vi "Unload.vi"(8 "error in (no error)":errorcluster, 10 "Unload":string, 11 "Sequencing in":refnum<class "Sequencing.lvclass">) -> (0 "error out":errorcluster, 3 "Sequencing out":refnum<class "Sequencing.lvclass">)   [LabVIEW 2020, in "VolatusSeq.lvlib" / "Sequencing.lvclass"]
uses:
  Sequencing.lvclass
  Sequencing.lvclass/Sequencing.ctl
  Sequence/Sequence.lvclass
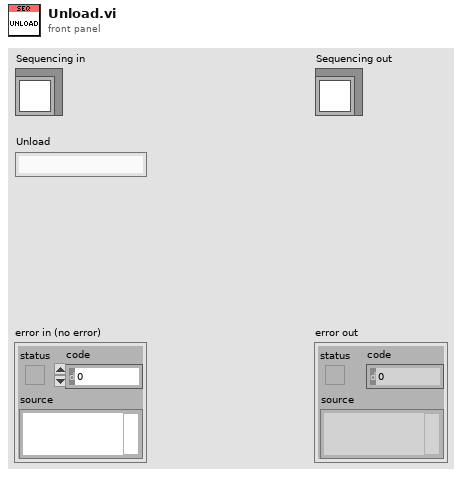
[diagram p1: front panel]
types:
  T1 = typedef "VolatusSeq.lvlib/Sequence Status.ctl" = cluster{"Name":string, "State":string, "Time":T2, "Running":bool}
  T2 = typedef "VolatusSeq.lvlib/Sequence Time.ctl" = cluster{"Abort":bool, "Seq Time":dbl, "State Time":dbl, "Wall Time":dbl}
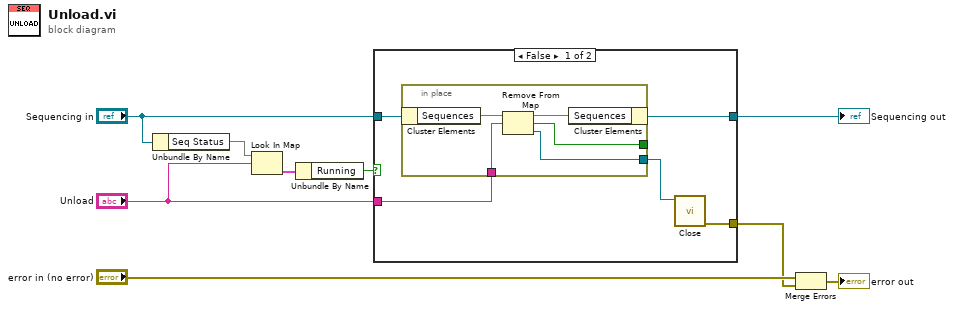
[diagram p0: block diagram]
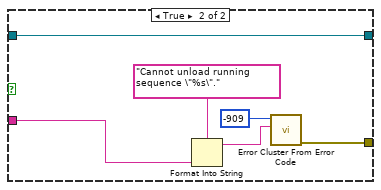
[diagram p2: hidden frame]
diagram:
  n1 = Unbundle By Name("Sequencing in") -> ("Seq Status"=w5:map{string, T1})
  n2 = Look In Map(map=w5, key="Unload") -> (value=w4:T1)  [unwired: 1 in, 1 out]
  n3 = Unbundle By Name(w4) -> ("Running"=w3:bool)
  n4 = case shown="False" w3 {
    tunnel: [w14 w25] -> w7
    tunnel: "Unload" -> [w10 w23]
    tunnel: "Sequencing in" -> [w13 w20]
    tunnel: [w12 w20] -> w2
    frame False {
      n5 = in-place {
        in-place-border: [w17] -> w11
        in-place-border: [w16] -> _
        in-place-border: w10 -> [w15]
        n6 = in-place-cluster #1(w13) -> ("Sequences"=w19:map{string, refnum<class "Sequence.lvclass">})
        n7 = Remove From Map(10:w15, 11:w19) -> (1:w17:refnum<class "Sequence.lvclass">, 2:w16:bool, 3:w18:map{string, refnum<class "Sequence.lvclass">})
        n8 = in-place-cluster #1("Sequences"=w18) -> (w12:refnum<class "Sequencing.lvclass">)
      }
      n9 = call "Close.vi"("Sequence in"=w11) -> ("error out"=w14:errorcluster)  [unwired: 9 in, 1 out]
    }
    frame True {
      n10 = Format Into String(format string="Cannot unload running sequence \"%s\".", w23) -> (resulting string=w21:string)  [unwired: 2 in, 1 out]
      n11 = call <vilib>:"Error Cluster From Error Code.vi"("error message (\"\")"=w21, "error code (0)"=-909) -> ("error out"=w25:errorcluster)  [unwired: 7 in]
    }
  }
  "Sequencing out" <- w2
  n12 = Merge Errors("error in (no error)", w7) -> (→"error out":errorcluster)
